vi "GDSString_ParseTextBasedCode.vi"(8 "error in (no error)":errorcluster, 11 "TextIn":string="public interface IGoldMembership\n    {\n        decimal GetDiscount(decimal amount);\n        bool IsShippingFree { get; set; }\n    }\n \npublic class GoldMembership : IGoldMembership\n    {\n        public GoldMembership(string userName)\n        {\n            // get gold member profile of this user\n \n            IsShippingFree = true;\n        }\n \n        public bool IsShippingFree { get; set; }\n \n        public decimal GetDiscount(decimal amount)\n        {\n            decimal discount = 100;\n \n            //calculate discount\n \n            return discount;\n        }\n    }\n \npublic class NullGoldMembership : IGoldMembership\n    {\n        public NullGoldMembership()\n        {\n            IsShippingFree = false;\n        }\n \n        public decimal GetDiscount(decimal amount)\n        {\n            return 0;\n        }\n \n        public bool IsShippingFree { get; set; }\n    }\n \npublic class GoldMembershipController\n    {\n        public static IGoldMembership GetProfile(Account account)\n        {\n            // if this account has gold membership \n            // return profile else return null\n \n            if (account.Type == \"GoldMember\")\n            {\n                return new GoldMembership(account.UserName);\n            }\n            else\n            {\n                return new NullGoldMembership();\n            }\n        }\n    }\n") -> (0 "error out":errorcluster, 1 "EnumsOusideClass":T1[](array[typedef])=[{"Name"="Orientation", "AccessScope"=enum."public", "Modifiers"=[], "Items"=["TOP", "LEFT"], "Documentation"=""}, {"Name"="Range", "AccessScope"=enum."public", "Modifiers"=[], "Items"=["Max", "Min"], "Documentation"=""}, {"Name"="CarOptions", "AccessScope"=enum."public", "Modifiers"=[], "Items"=["SunRoof", "Spoiler", "FogLights", "TintedWindows"], "Documentation"=""}], 2 "StructsOusideClass":T4[](array[typedef])=[{"Name"="", "AccessScope"=enum."public", "Modifiers"=[], "Items"=[], "Documentation"=""}], 3 "Classes":T7[](array[typedef])=[{"ClassName"="EmailErrorHandler", "AccessScope"=enum."public", "Modifiers"=[], "ClassDocumentation"="public", "Methods"=[{"ReturnType"={"Name"="", "DataType"=enum."UINT8", "ArrayDim"=0, "CtrlPath"=path "", "DataTypeString"="", "AccessScope"=enum."public", "InitialData"=variant}, "MethodName"="", "AccessScope"=enum."public", "Modifiers"=[], "MethodDocumentation"="", "MethodContent"="", "MethodArguments"=[], "GetProperty"={"Active"=FALSE, "AccessScope"=enum."public", "Code"=""}, "SetProperty"={"Active"=FALSE, "AccessScope"=enum."public", "Code"=""}}, {"ReturnType"={"Name"="", "DataType"=enum."UINT8", "ArrayDim"=0, "CtrlPath"=path "", "DataTypeString"="", "AccessScope"=enum."public", "InitialData"=variant}, "MethodName"="", "AccessScope"=enum."public", "Modifiers"=[], "MethodDocumentation"="", "MethodContent"="", "MethodArguments"=[], "GetProperty"={"Active"=FALSE, "AccessScope"=enum."public", "Code"=""}, "SetProperty"={"Active"=FALSE, "AccessScope"=enum."public", "Code"=""}}, {"ReturnType"={"Name"="", "DataType"=enum."UINT8", "ArrayDim"=0, "CtrlPath"=path "", "DataTypeString"="", "AccessScope"=enum."public", "InitialData"=variant}, "MethodName"="", "AccessScope"=enum."public", "Modifiers"=[], "MethodDocumentation"="", "MethodContent"="", "MethodArguments"=[], "GetProperty"={"Active"=FALSE, "AccessScope"=enum."public", "Code"=""}, "SetProperty"={"Active"=FALSE, "AccessScope"=enum."public", "Code"=""}}, {"ReturnType"={"Name"="", "DataType"=enum."UINT8", "ArrayDim"=0, "CtrlPath"=path "", "DataTypeString"="", "AccessScope"=enum."public", "InitialData"=variant}, "MethodName"="", "AccessScope"=enum."public", "Modifiers"=[], "MethodDocumentation"="", "MethodContent"="", "MethodArguments"=[], "GetProperty"={"Active"=FALSE, "AccessScope"=enum."public", "Code"=""}, "SetProperty"={"Active"=FALSE, "AccessScope"=enum."public", "Code"=""}}], "ParentClasses"=[{"ClassName"="IErrorHandler", "ClassType"=enum."Undefined"}], "ClassType"=enum."Class", "Owner"="", "OwnerType"=enum."NoOwner", "Generics"=[], "Attributes"=[{"Name"="settings", "DataType"=enum."Other", "ArrayDim"=0, "CtrlPath"=path "", "DataTypeString"="EmailErrorHandlerParms", "AccessScope"=enum."private", "InitialData"=variant(string "")}], "Enums"=[], "Structs"=[]}, {"ClassName"="EmailErrorHandlerParms", "AccessScope"=enum."public", "Modifiers"=[], "ClassDocumentation"="", "Methods"=[{"ReturnType"={"Name"="", "DataType"=enum."UINT8", "ArrayDim"=0, "CtrlPath"=path "", "DataTypeString"="", "AccessScope"=enum."public", "InitialData"=variant}, "MethodName"="", "AccessScope"=enum."public", "Modifiers"=[], "MethodDocumentation"="", "MethodContent"="", "MethodArguments"=[], "GetProperty"={"Active"=FALSE, "AccessScope"=enum."public", "Code"=""}, "SetProperty"={"Active"=FALSE, "AccessScope"=enum."public", "Code"=""}}, {"ReturnType"={"Name"="", "DataType"=enum."UINT8", "ArrayDim"=0, "CtrlPath"=path "", "DataTypeString"="", "AccessScope"=enum."public", "InitialData"=variant}, "MethodName"="", "AccessScope"=enum."public", "Modifiers"=[], "MethodDocumentation"="", "MethodContent"="", "MethodArguments"=[], "GetProperty"={"Active"=FALSE, "AccessScope"=enum."public", "Code"=""}, "SetProperty"={"Active"=FALSE, "AccessScope"=enum."public", "Code"=""}}, {"ReturnType"={"Name"="", "DataType"=enum."UINT8", "ArrayDim"=0, "CtrlPath"=path "", "DataTypeString"="", "AccessScope"=enum."public", "InitialData"=variant}, "MethodName"="", "AccessScope"=enum."public", "Modifiers"=[], "MethodDocumentation"="", "MethodContent"="", "MethodArguments"=[], "GetProperty"={"Active"=FALSE, "AccessScope"=enum."public", "Code"=""}, "SetProperty"={"Active"=FALSE, "AccessScope"=enum."public", "Code"=""}}, {"ReturnType"={"Name"="", "DataType"=enum."UINT8", "ArrayDim"=0, "CtrlPath"=path "", "DataTypeString"="", "AccessScope"=enum."public", "InitialData"=variant}, "MethodName"="", "AccessScope"=enum."public", "Modifiers"=[], "MethodDocumentation"="", "MethodContent"="", "MethodArguments"=[], "GetProperty"={"Active"=FALSE, "AccessScope"=enum."public", "Code"=""}, "SetProperty"={"Active"=FALSE, "AccessScope"=enum."public", "Code"=""}}, {"ReturnType"={"Name"="", "DataType"=enum."UINT8", "ArrayDim"=0, "CtrlPath"=path "", "DataTypeString"="", "AccessScope"=enum."public", "InitialData"=variant}, "MethodName"="", "AccessScope"=enum."public", "Modifiers"=[], "MethodDocumentation"="", "MethodContent"="", "MethodArguments"=[], "GetProperty"={"Active"=FALSE, "AccessScope"=enum."public", "Code"=""}, "SetProperty"={"Active"=FALSE, "AccessScope"=enum."public", "Code"=""}}], "ParentClasses"=[], "ClassType"=enum."Class", "Owner"="EmailErrorHandler", "OwnerType"=enum."Class", "Generics"=[], "Attributes"=[], "Enums"=[], "Structs"=[]}])   [LabVIEW 2020]
uses:
  GDSString_ClassDescriptionType.ctl
  GDSString_AccessScopeModifierType.ctl
  GDSString_ModifierType.ctl
  GDSString_MethodDescriptionType.ctl
  CommonVIs/CommonVIs_AttributeType.ctl
  CommonVIs/CommonVIs_AttributeDataType.ctl
  CommonVIs/CommonVIs_PropertyType.ctl
  GDSString_ClassParentType.ctl
  GDSString_ClassType.ctl
  GDSString_ClassOwnerType.ctl
  CommonVIs/CommonVIs_EnumType.ctl
  CommonVIs/CommonVIs_StructType.ctl
panel:
  # "using System;\n\nnamespace TutlaneExamples\n{\n    class Users\n    {\n       // Declare an array\n       private string[] arr = new string[3];\n       // Define the indexer\n       public string this[int i]\n       {\n          get { return arr[i]; }\n          set { arr[i] = value; }\n       }\n    }\n    class Program\n    {\n       static void Main(string[] args)\n       {\n          Users ulist = new Users();\n          ulist[0] = \"Suresh Dasari\";\n          ulist[1] = \"Rohini Alavala\";\n          ulist[2] = \"Trishika Dasari\";\n          for (int i = 0; i < 3; i++)\n          {\n             Console.WriteLine(ulist[i]);\n          }\n          Console.ReadLine();\n       }\n    }\n}"
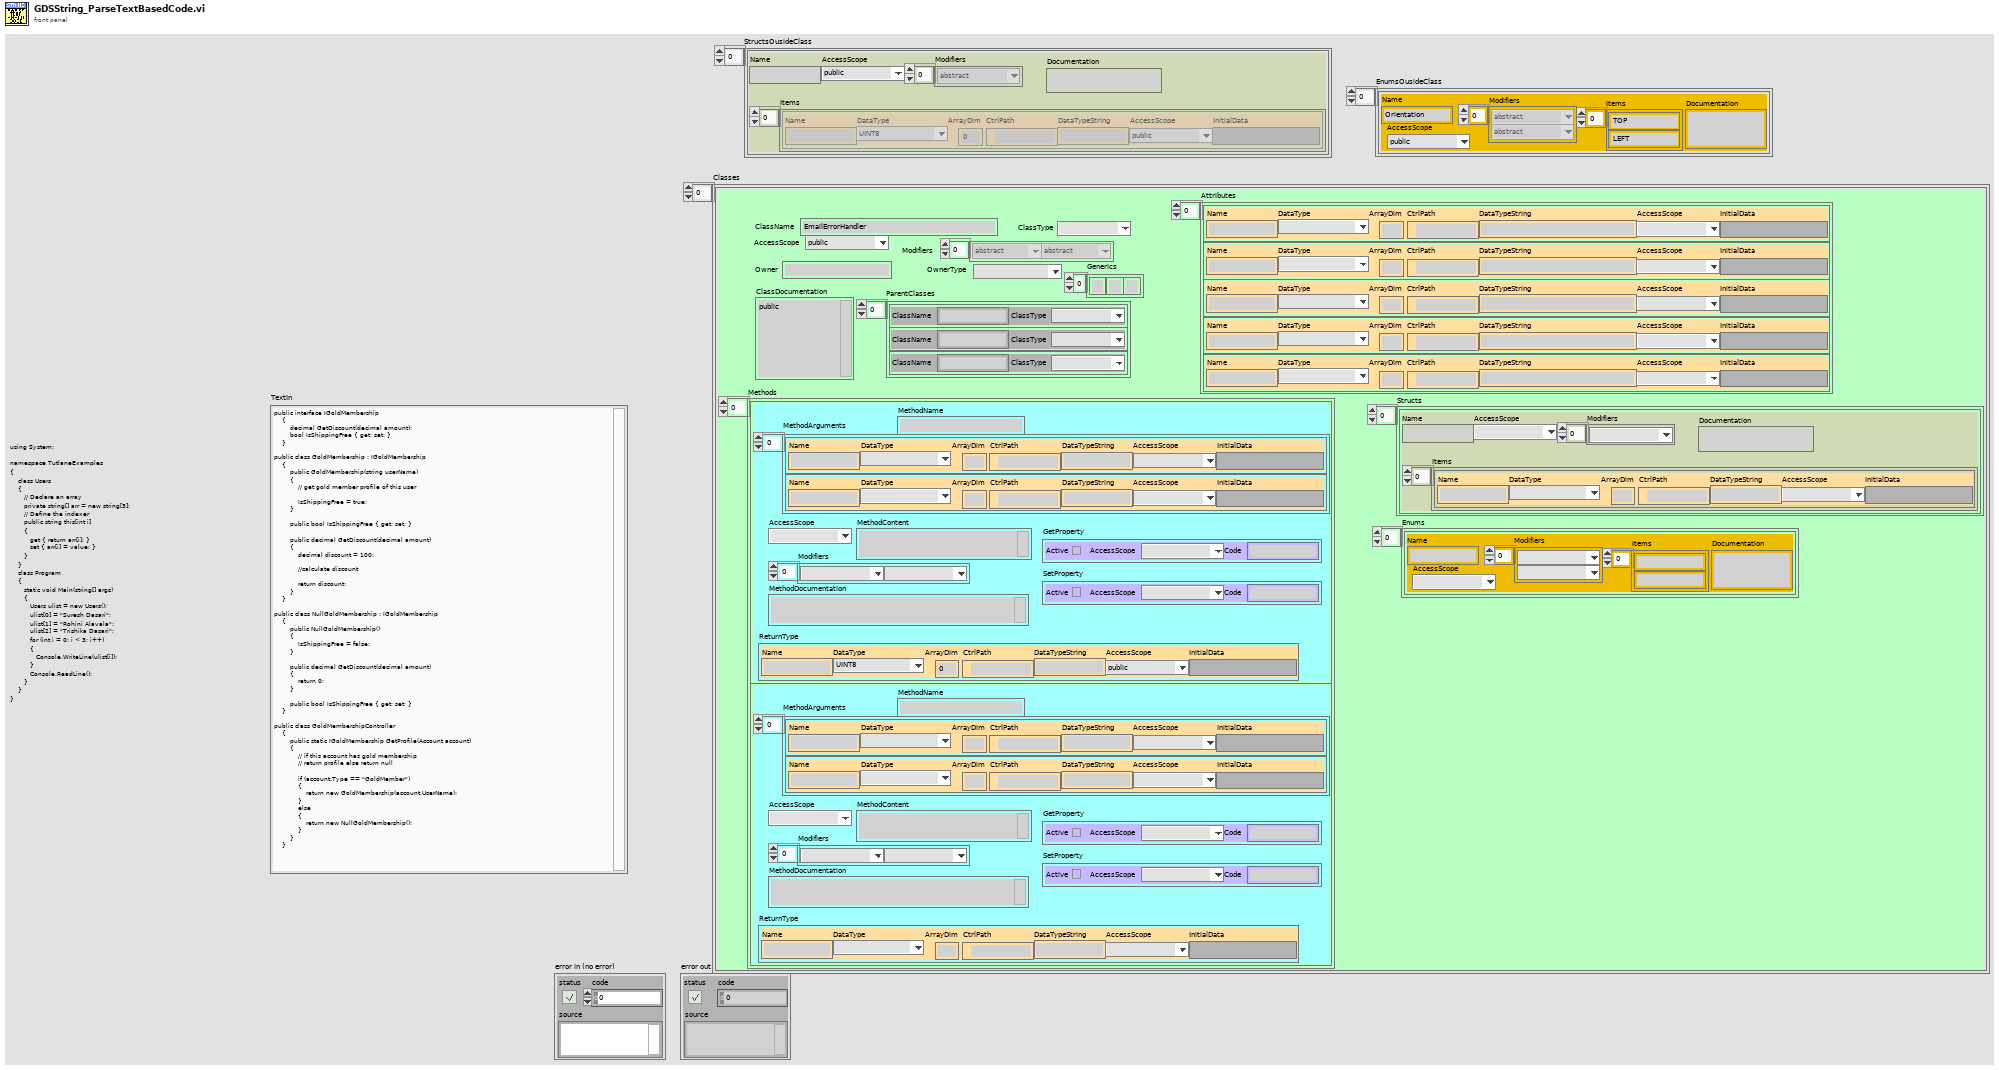
[diagram p1: front panel]
types:
  T1 = typedef "CommonVIs_EnumType.ctl" = cluster{"Name":string, "AccessScope":T2, "Modifiers":T3[], "Items":string[], "Documentation":string}
  T2 = typedef "GDSString_AccessScopeModifierType.ctl" = enum16{"public", "private", "protected", "internal"}
  T3 = typedef "GDSString_ModifierType.ctl" = enum16{"abstract", "static", "final", "synchronized", "strictfp", "async", "const", "event", "extern", "new", "native ", "override", "partial", "readonly", "sealed", "unsafe", "virtual", "volatile"}
  T4 = typedef "CommonVIs_StructType.ctl" = cluster{"Name":string, "AccessScope":T2, "Modifiers":T3[], "Items":T5[], "Documentation":string}
  T5 = typedef "CommonVIs_AttributeType.ctl" = cluster{"Name":string, "DataType":T6, "ArrayDim":i32, "CtrlPath":path, "DataTypeString":string, "AccessScope":T2, "InitialData":variant}
  T6 = typedef "CommonVIs_AttributeDataType.ctl" = enum16{"UINT8", "INT8", "UINT16", "INT16", "UINT32", "INT32", "UINT64", "INT64", "SGL", "DBL", "EXT", "CSG", "CDB", "CXT", "TimeStamp", "STRING", "PATH", "BOOL", "ENUM", "RefNum", "VIRefNum", "LabVIEW Class", "Cluster", "Variant", "TypeDef", "Waveform", "LabVIEW Object", "Other", "void", "Set", "Map"}
  T7 = typedef "GDSString_ClassDescriptionType.ctl" = cluster{"ClassName":string, "AccessScope":T2, "Modifiers":T3[], "ClassDocumentation":string, "Methods":T8[], "ParentClasses":T10[], "ClassType":T11, "Owner":string, "OwnerType":T12, "Generics":string[], "Attributes":T5[], "Enums":T1[], "Structs":T4[]}
  T8 = typedef "GDSString_MethodDescriptionType.ctl" = cluster{"ReturnType":T5, "MethodName":string, "AccessScope":T2, "Modifiers":T3[], "MethodDocumentation":string, "MethodContent":string, "MethodArguments":T5[], "GetProperty":T9, "SetProperty":T9}
  T9 = typedef "CommonVIs_PropertyType.ctl" = cluster{"Active":bool, "AccessScope":T2, "Code":string}
  T10 = typedef "GDSString_ClassParentType.ctl" = cluster{"ClassName":string, "ClassType":T11}
  T11 = typedef "GDSString_ClassType.ctl" = enum16{"Undefined", "Class", "Interface"}
  T12 = typedef "GDSString_ClassOwnerType.ctl" = enum16{"NoOwner", "Class", "Package/NameSpace"}
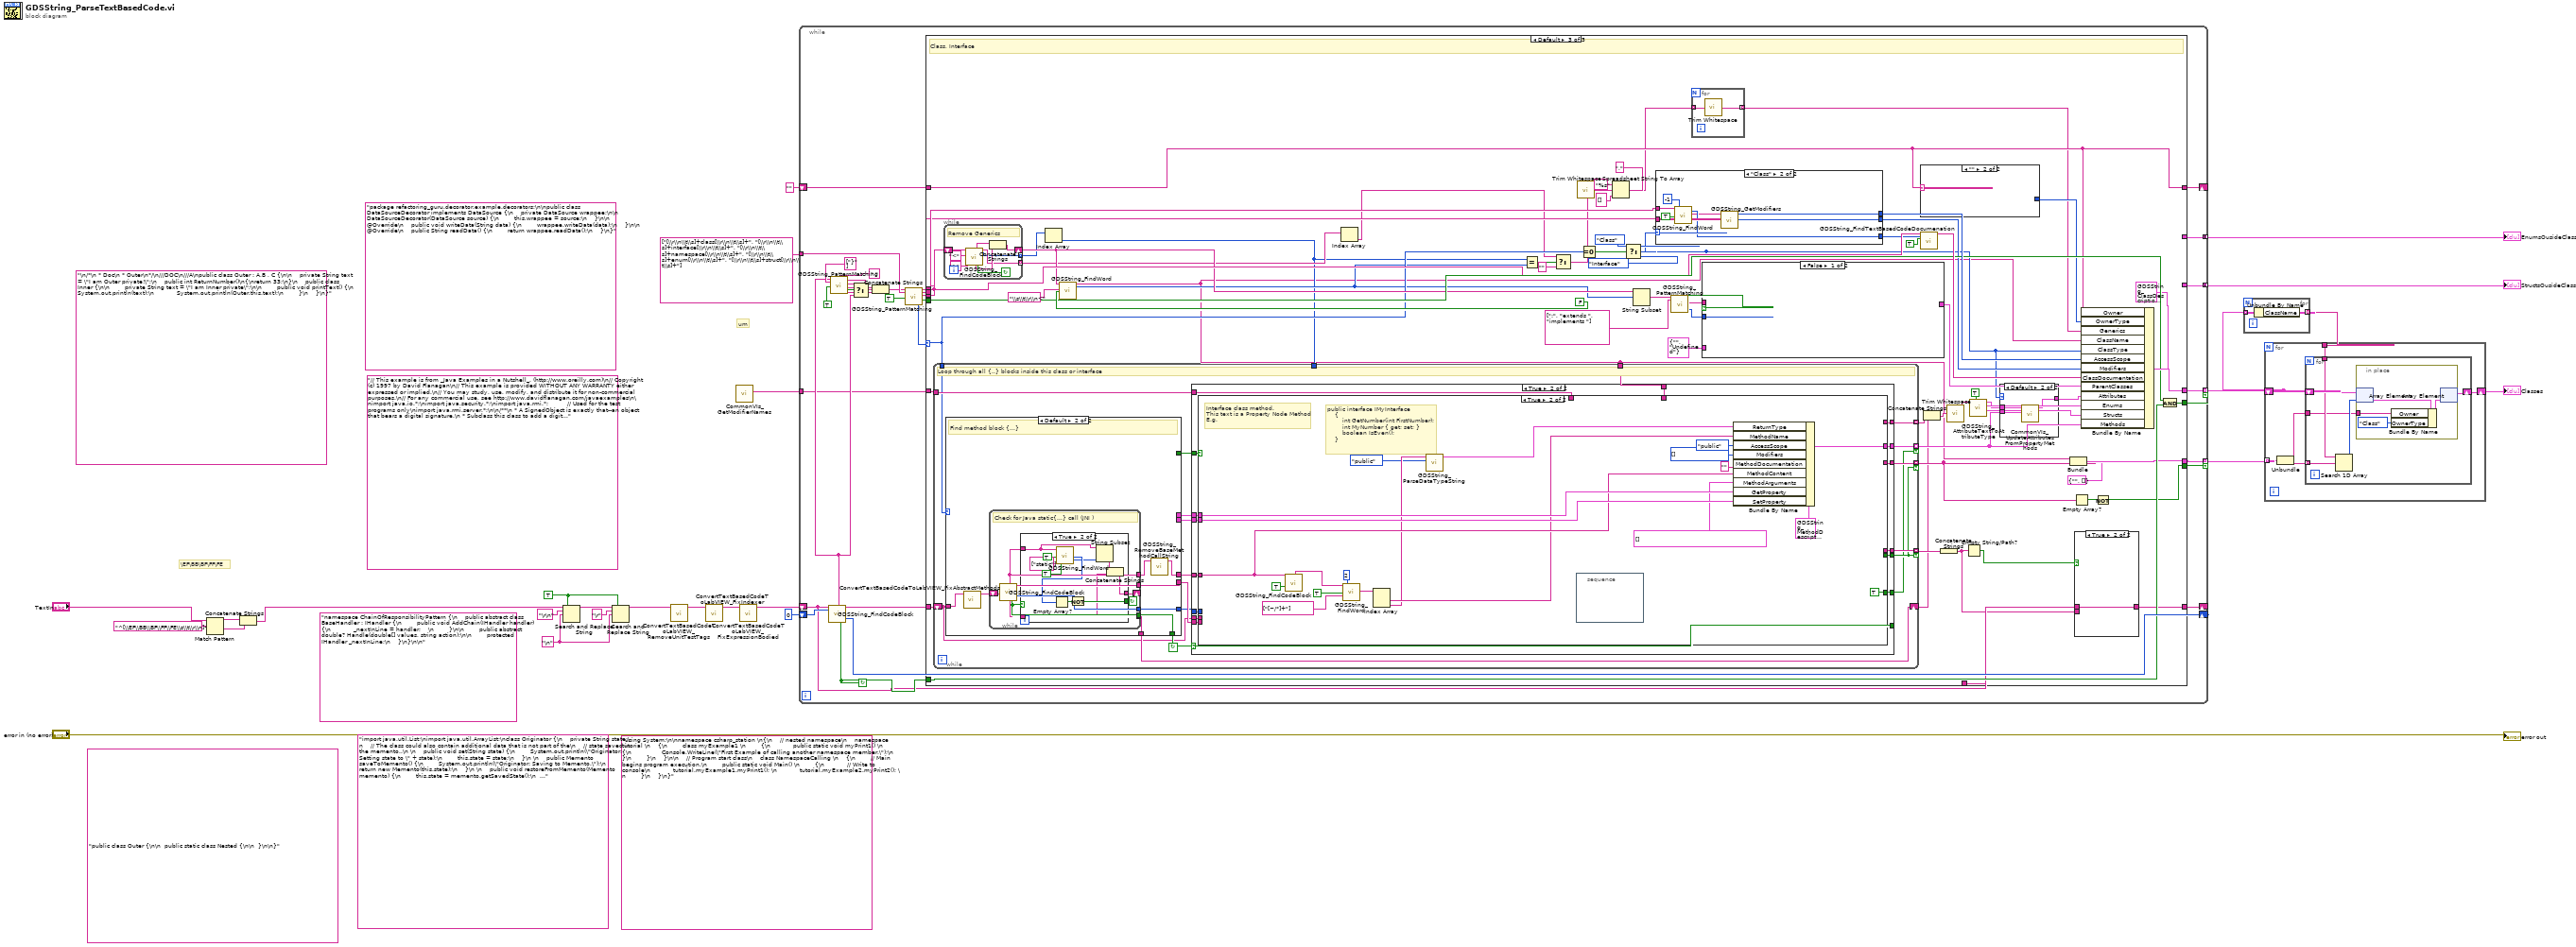
[diagram p0: block diagram]
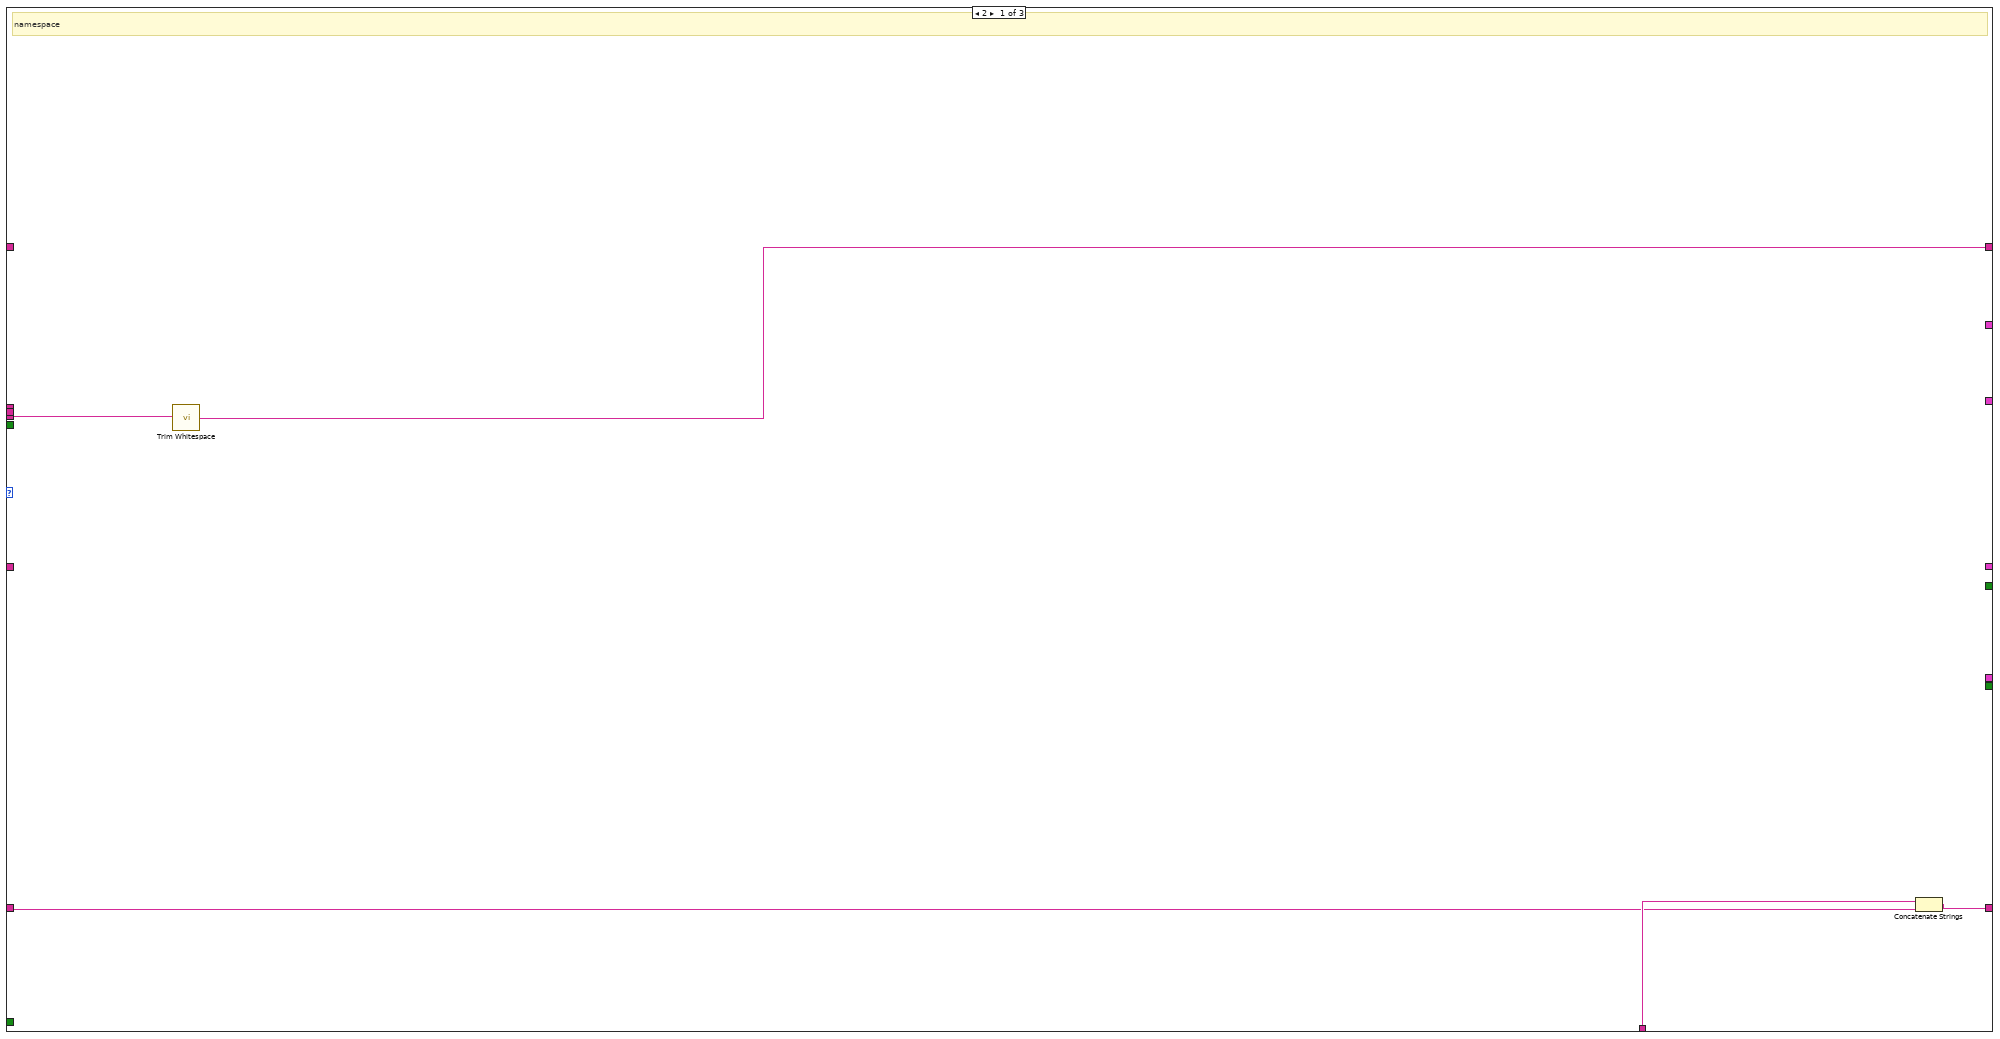
[diagram p2: hidden frame]
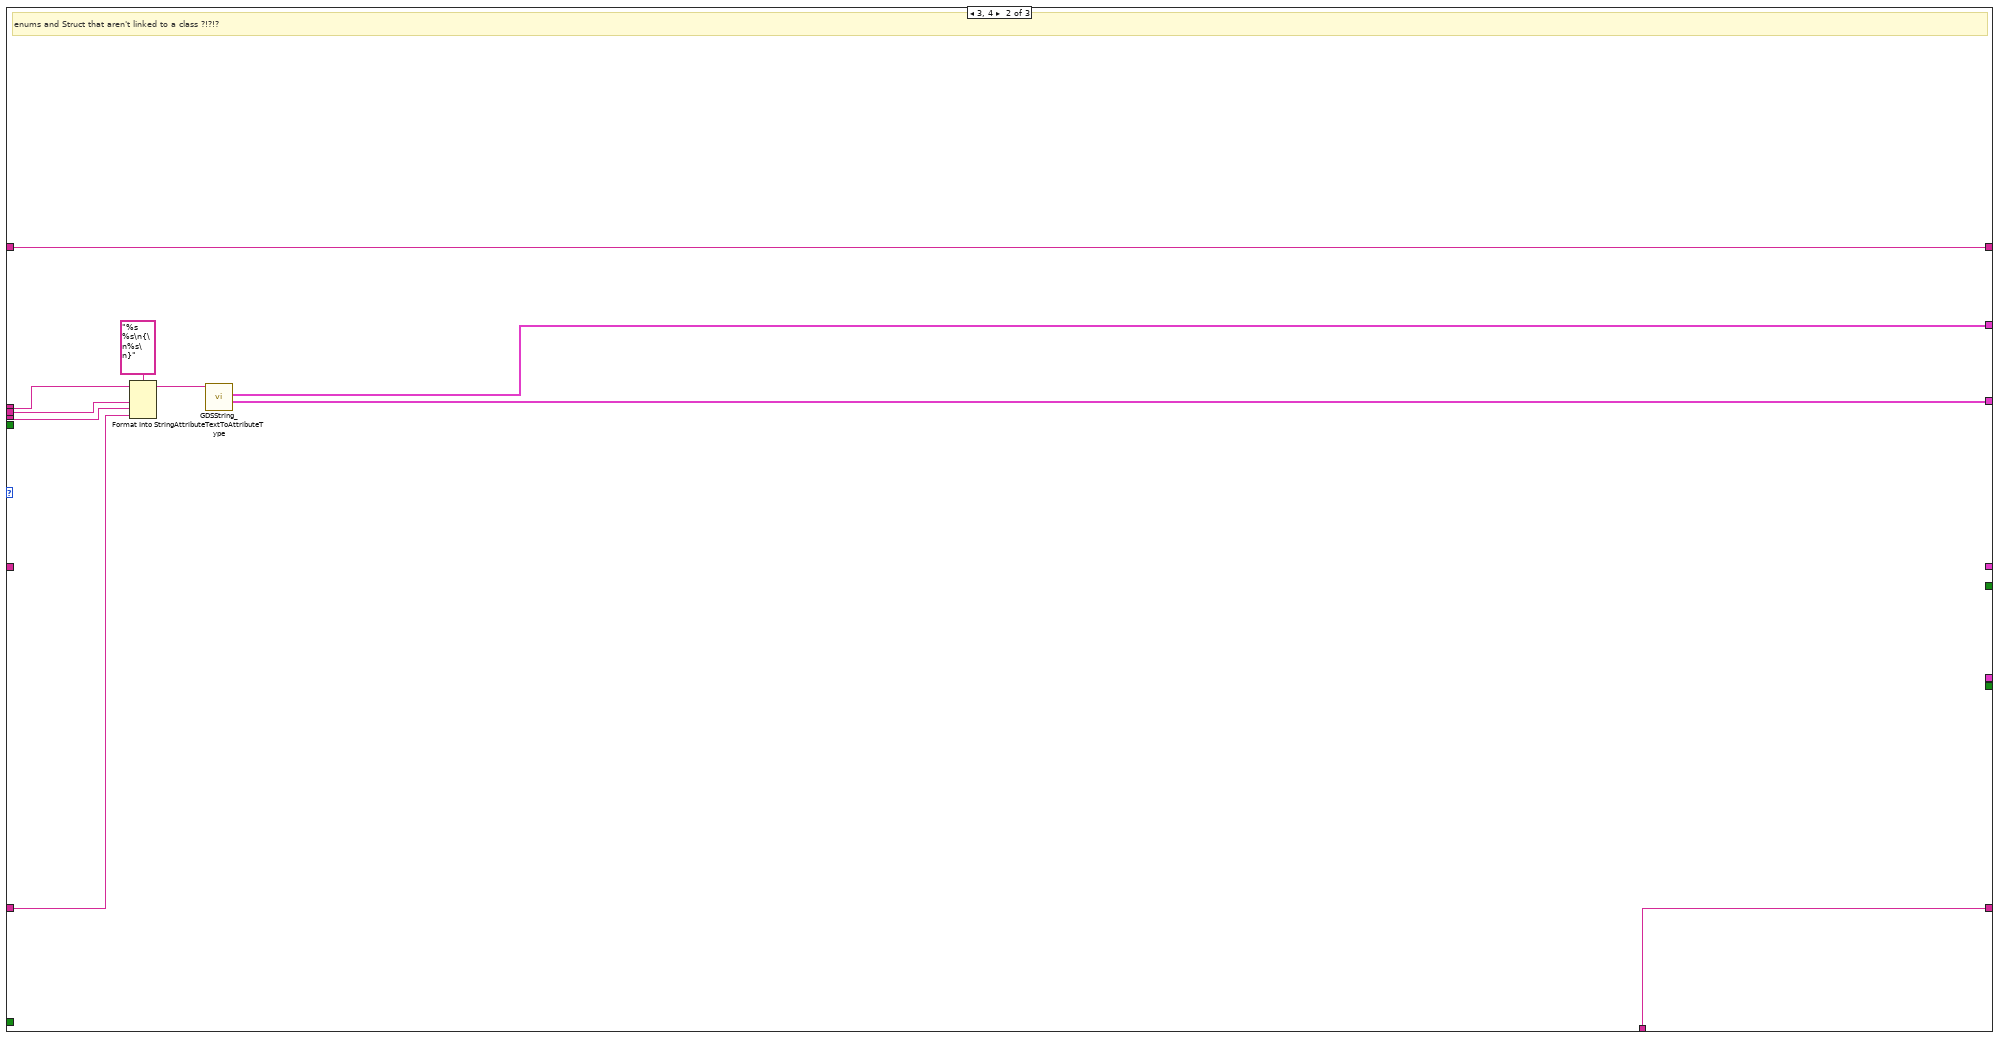
[diagram p3: hidden frame]
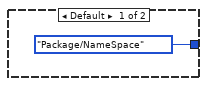
[diagram p5: hidden frame]
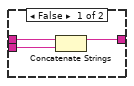
[diagram p6: hidden frame]
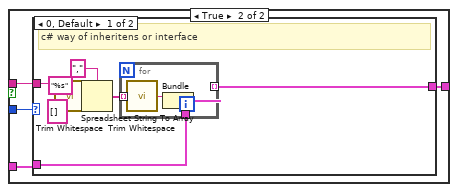
[diagram p7: hidden frame]
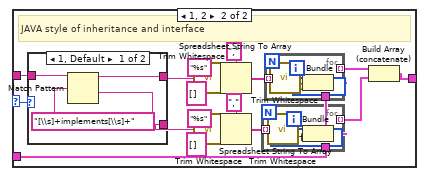
[diagram p8: hidden frame]
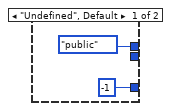
[diagram p10: hidden frame]
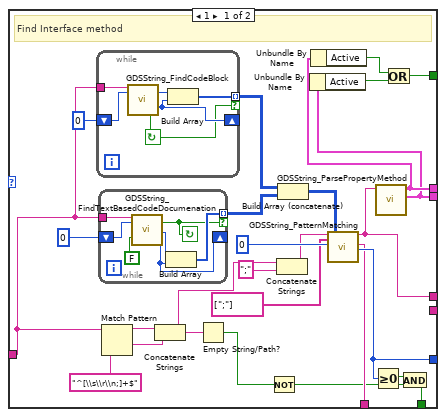
[diagram p11: hidden frame]
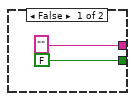
[diagram p12: hidden frame]
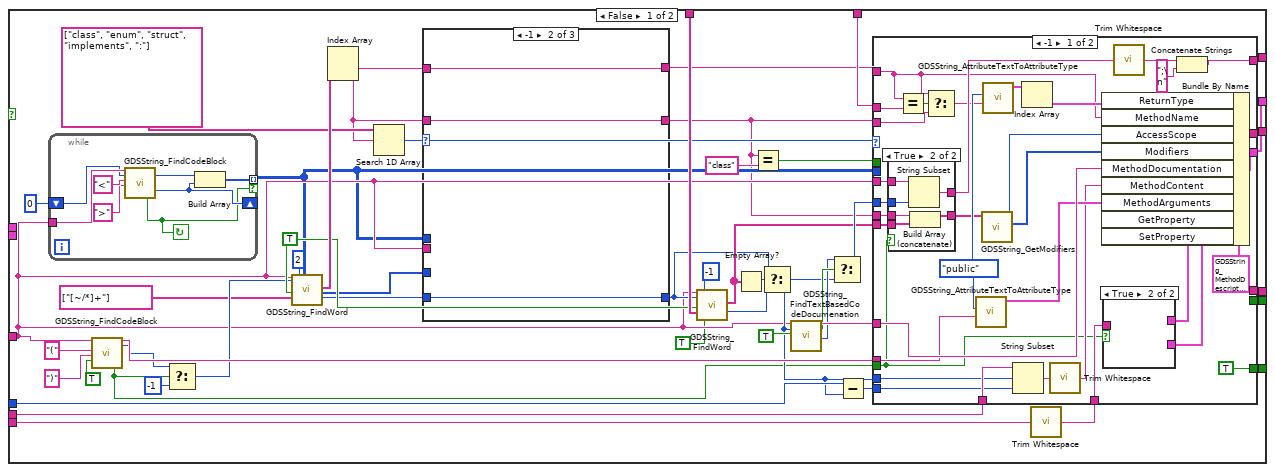
[diagram p14: hidden frame]
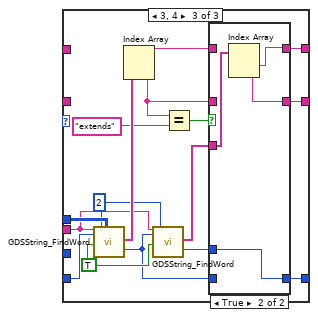
[diagram p16: hidden frame]
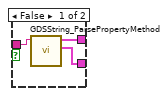
[diagram p19: hidden frame]
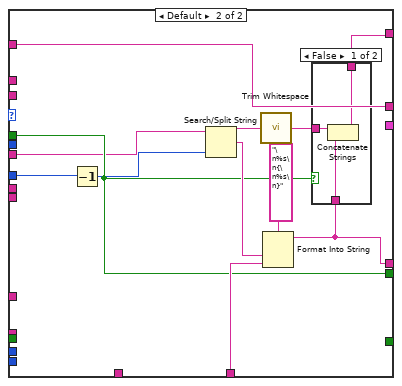
[diagram p20: hidden frame]
diagram:
  (unwired) "namespace ChainOfResponsibilityPattern {\n    public abstract class BaseHandler : IHandler {\n        public void AddChain(IHandler handler) {\n            _nextInLine = handler;    \n        }\n\n        public abstract double? Handle(double[] values, string action);\n\n        protected IHandler _nextInLine;\n    }\n}\n\n" ("search string")
  (unwired) "package refactoring_guru.decorator.example.decorators;\n\npublic class DataSourceDecorator implements DataSource {\n    private DataSource wrappee;\n\n    DataSourceDecorator(DataSource source) {\n        this.wrappee = source;\n    }\n\n    @Override\n    public void writeData(String data) {\n        wrappee.writeData(data);\n    }\n\n    @Override\n    public String readData() {\n        return wrappee.readData();\n    }\n}" ("text")
  (unwired) "using System;\n\nnamespace csharp_station \n{\n    // nested namespace\n    namespace tutorial \n    {\n        class myExample1 \n        {\n            public static void myPrint1() \n            {\n                Console.WriteLine(\"First Example of calling another namespace member.\");\n            }\n        }\n    }\n\n    // Program start class\n    class NamespaceCalling \n    {\n        // Main begins program execution.\n        public static void Main() \n        {\n            // Write to console\n            tutorial.myExample1.myPrint1(); \n            tutorial.myExample2.myPrint2(); \n        }\n    }\n}" ("text")
  (unwired) "public class Outer {\n\n  public static class Nested {\n\n  }\n\n}" ("text")
  (unwired) "import java.util.List;\nimport java.util.ArrayList;\nclass Originator {\n    private String state;\n    // The class could also contain additional data that is not part of the\n    // state saved in the memento..\n \n    public void set(String state) {\n        System.out.println(\"Originator: Setting state to \" + state);\n        this.state = state;\n    }\n \n    public Memento saveToMemento() {\n        System.out.println(\"Originator: Saving to Memento.\");\n        return new Memento(this.state);\n    }\n \n    public void restoreFromMemento(Memento memento) {\n        this.state = memento.getSavedState();\n        System.out.println(\"Originator: State after restoring from Memento: \" + state);\n    }\n \n    public static class Memento {\n        private final String state;\n \n        public Memento(String stateToSave) {\n            state = stateToSave;\n        }\n \n        public String getSavedState() {\n            return state;\n        }\n    }\n}\n \nclass Caretaker {\n    public static void main(String[] args) {\n        List<Originator.Memento> savedStates = new ArrayList<Originator.Memento>();\n \n        Originator originator = new Originator();\n        originator.set(\"State1\");\n        originator.set(\"State2\");\n        savedStates.add(originator.saveToMemento());\n        originator.set(\"State3\");\n        // We can request multiple mementos, and choose which one to roll back to.\n        savedStates.add(originator.saveToMemento());\n        originator.set(\"State4\");\n \n        originator.restoreFromMemento(savedStates.get(1));   \n    }\n}" ("text")
  (unwired) "// This example is from _Java Examples in a Nutshell_. (http://www.oreilly.com)\n// Copyright (c) 1997 by David Flanagan\n// This example is provided WITHOUT ANY WARRANTY either expressed or implied.\n// You may study, use, modify, and distribute it for non-commercial purposes.\n// For any commercial use, see http://www.davidflanagan.com/javaexamples\n\nimport java.io.*;\nimport java.security.*;\nimport java.rmi.*;          // Used for the test programs only\nimport java.rmi.server.*;\n\n/**\n * A SignedObject is exactly that--an object that bears a digital signature.\n * Subclass this class to add a digital signature to any class you want.\n * Note, however, that the signature is computed using serialization, so only\n * the serializable, non-transient fields of a subclass are included in\n * the signature computation.\n **/\npublic class SignedObject implements Serializable {\n  protected String signername;               // Who is doing the signing\n  protected String algorithm;                // What algorithm to use.\n  private byte[] signature;                  // The bytes of the signature\n  transient private boolean signing = false; // A flag used below.\n\n  /**\n   * This method computes a digital signature for the current state of the\n   * object, excluding the signature-related state of this class.\n   * That is, the signature is based only on the state of the subclasses.\n   * The arguments specify who is signing the object, and what digital \n   * signature algorithm to use.\n   * \n   * Note that no other threads should be modifying the object while\n   * this computation is being performed.  If a subclass will be used in a \n   * multi-threaded environment, this means that methods of the subclass\n   * that modify its state should be synchronized like this one is.\n   **/\n  public synchronized void sign(String signername, String algorithm) \n       throws IOException, InvalidKeyException, \n         SignatureException, NoSuchAlgorithmException \n  {\n    // Save the arguments for use by verify()\n    this.signername = signername;\n    this.algorithm = algorithm;\n\n    // Get a Signature object to compute the signature with\n    Signature s = Signature.getInstance(algorithm);\n\n    // Get a Signer object representing the signer\n    Signer signer = \n      (Signer)IdentityScope.getSystemScope().getIdentity(signername);\n\n    // Initialize the Signature object using the PrivateKey of the Signer\n    s.initSign(signer.getPrivateKey());\n\n    // Create an ObjectOutputStream that writes its output to a \n    // ByteArrayStream.  This is how we capture the state of the object\n    // so that it can be signed.\n    ByteArrayOutputStream bout = new ByteArrayOutputStream();\n    ObjectOutputStream out = new ObjectOutputStream(bout);\n\n    // Now serialize the object, capturing its state.  We have to set a flag\n    // before we do this, so that the signer name, algorithm, and signature\n    // itself are not included in this serialized state.  See writeObject()\n    // below to see how this works.\n    signing = true;\n    out.writeObject(this);\n    signing = false;\n\n    // Now tell the Signature object about the bytes of serialized state\n    // that were stored by the ByteArrayOutputStream\n    s.update(bout.toByteArray());\n\n    // And finally, compute the signature\n    this.signature = s.sign();\n  }\n\n  /** A simpler version of sign(), that defaults to using the DSA algorithm */\n  public synchronized void sign(String signername) \n       throws IOException, InvalidKeyException, \n         SignatureException, NoSuchAlgorithmException {\n    sign(signername, \"DSA\");\n  }\n\n  /**\n   * This method verifies the signature of any SignedObject subclass.\n   * It works much like the sign() method, and is also synchronized.\n   **/\n  public synchronized boolean verify() \n       throws IOException, InvalidKeyException,\n         SignatureException, NoSuchAlgorithmException\n  {\n    // Make sure the object is actually signed.\n    if (signature == null) \n      throw new SignatureException(\"Object is not signed\");\n\n    // Get the signature, signer and public key, and initialize, like above,\n    // except that this time use a PublicKey instead of a PrivateKey\n    Signature s = Signature.getInstance(algorithm);\n    Identity signer = \n      (Identity)IdentityScope.getSystemScope().getIdentity(signername);\n    s.initVerify(signer.getPublicKey());\n\n    // Create streams and capture the current state of the object \n    // (excluding the signature bytes themselves) in a byte array\n    ByteArrayOutputStream bout = new ByteArrayOutputStream();\n    ObjectOutputStream out = new ObjectOutputStream(bout);\n    signing = true;\n    out.writeObject(this);\n    signing = false;\n\n    // Pass state of the object to the Signature, and verify the stored\n    // signature bytes against that state.  Return the result of verification.\n    s.update(bout.toByteArray());\n    return s.verify(this.signature);\n  }\n\n  /**\n   * When the contents of the object change, the signature becomes invalid.\n   * When this happens, the signature should be erased, because validation\n   * is guaranteed to fail.\n   **/\n  public void removeSignature() { \n    signature = null; signername = null; algorithm = null; \n  }\n\n  /**\n   * This method is invoked to allow custom serialization.\n   * We only write out our signature-related state when we are not computing\n   * or verifying a signature.  When we are computing or verifying, only our\n   * subclass state gets written out.  If we don't do this, verification will\n   * fail because the signature[] array will obviously be different on\n   * verification than it is when the signature is generated.\n   **/\n  private void writeObject(ObjectOutputStream out) throws IOException {\n    if (!signing) out.defaultWriteObject();\n  }\n}\n\n/**\n * This class is a simple SignedObject subclass.\n * This and the following interface and classes are used to test SignedObject.\n **/\nclass SignedString extends SignedObject {\n  public String s;\n  public SignedString(String s) { this.s = s; }\n}\n\n/**\n * This interface extends Remote.  It is part of an RMI example using our\n * SignedString class above.\n **/\ninterface RemoteSignedString extends Remote {\n  public SignedString getString() throws RemoteException;\n}\n\n/**\n * This is a simple RMI server class and a program to start and register the\n * server.  The server creates a SignedString object, signs it, and then \n * exports it to clients through the RemoteSignedString getString() method.\n **/\nclass SignedStringServer extends UnicastRemoteObject \n                         implements RemoteSignedString \n{\n  SignedString s;  // The state of the server object\n\n  /** The constructor.  Initialize the SignedString */\n  public SignedStringServer(SignedString s) throws RemoteException {this.s=s;}\n\n  /** This is the remote method exported by the server */\n  public SignedString getString() throws RemoteException { return s; }\n  \n  /** The main program that creates and registers the server object */\n  public static void main(String[] args) \n       throws NoSuchAlgorithmException, InvalidKeyException, \n         IOException, SignatureException\n  {\n    SignedString ss = new SignedString(args[0]);         // create object\n    ss.sign(args[1]);                                    // sign it\n    SignedStringServer sss = new SignedStringServer(ss); // start server\n    Naming.rebind(\"SignedStringServer\", sss);            // register server\n    System.out.println(\"Ready for clients\");             // up and running!\n  }\n}\n\n/**\n * This class is a client that connects to a RemoteSignedString server and\n * calls the getString() method to obtain a SignedString.  It then verifies\n * the signature of the object that it has just downloaded over a network\n * from an entirely different Java VM.  The client takes an optional hostname\n * argument on the command line.\n **/\nclass SignedStringClient {\n  public static void main(String[] args)\n       throws NoSuchAlgorithmException, InvalidKeyException, \n         IOException, SignatureException, NotBoundException\n  {\n    // Look up the server\n    RemoteSignedString rss = \n      (RemoteSignedString) Naming.lookup(\"rmi://\" + \n                                         ((args.length>0)?args[0]:\"\") +\n                                         \"/SignedStringServer\"); \n\n    // Invoke a remote method of the server to get a SignedString\n    SignedString ss = rss.getString();\n\n    // Now verify the signature on that SignedString.\n    if (ss.verify()) System.out.println(\"Verified SignedString: \" + ss.s);\n    else System.out.println(\"SignedString failed verification\");\n  }\n}\n" ("text")
  w10 = TRUE ("replace all? (F)")
  w22 = "\n" ("search string")
  (unwired) "\n/*\n * Doc\n * Outer\n*/\n///DOC\n///A\npublic class Outer : A,B , C {\n\n    private String text = \"I am Outer private!\";\n    public int ReturnNumber()\n{\nreturn 33;\n}\n    public class Inner {\n\n        private String text = \"I am Inner private\";\n\n        public void printText() {\n            System.out.println(text);\n            System.out.println(Outer.this.text);\n        }\n    }\n}" ("text")
  # "\\EF\\BB\\BF\\FF\\FE"
  # "um"
  n1 = Match Pattern(string="TextIn", regular expression="^[\\EF\\BB\\BF\\FF\\FE\\s\\t\\r\\n]+") -> (before substring=w8:string, after substring=w7:string)  [unwired: 1 in, 2 out]
  n2 = Concatenate Strings(w8, w7) -> (w5:string)
  n3 = Search and Replace String(replace all?=w10, input string=w5, search string="\r\n", replace string=w22) -> (result string=w25:string)  [unwired: 4 in, 3 out]
  n4 = Search and Replace String(replace all?=w10, input string=w25, search string="\r", replace string=w22) -> (result string=w2:string)  [unwired: 4 in, 3 out]
  n5 = call "ConvertTextBasedCodeToLabVIEW_RemoveUnitTestTags.vi"("TextIn"=w2) -> ("TextOut"=w1:string)  [unwired: 10 in]
  n6 = call "ConvertTextBasedCodeToLabVIEW_FixIndexer.vi"("IndexerTextIn"=w1) -> ("MofifiedIndexerTextOut"=w4:string)  [unwired: 10 in]
  n7 = call "CommonVIs_GetModifierNames.vi"() -> ("AllModifiers"=w13:string[])  [unwired: 9 in, 2 out]
  n8 = call "ConvertTextBasedCodeToLabVIEW_FixExpressionBodied.vi"("Expression-bodiedTextIn"=w4) -> ("ModifiedExpression-bodiedTextOut"=w3:string)  [unwired: 10 in]
  n9 = while {
    tunnel: w13 -> [w39]
    shift-right: [w53] -> _
    shift-left: 0 ("GetNext-X_Words(1,-1=All)") -> [w54]
    tunnel: [w52] -> w19 mode=indexing if=w43
    shift-right: [w37] -> _
    shift-left: w3 -> [w38]
    tunnel: [w36] -> w20 mode=indexing if=w35
    tunnel: string[] ["[\\r\\n\\t\\s]+class[\\r\\n\\t\\s]+", "[\\r\\n\\t\\s]+interface[\\r\\n\\t\\s]+", "[\\r\\n\\t\\s]+namespace[\\r\\n\\t\\s]+", "[\\r\\n\\t\\s]+enum[\\r\\n\\t\\s]+", "[\\r\\n\\t\\s]+struct[\\r\\n\\t\\s]+"] -> [w34]
    shift-right: [w31] -> _
    shift-left: "" ("trimmed string") -> [w30]
    tunnel: [w27] -> w11 mode=concatenating
    tunnel: [w26] -> w12 mode=concatenating
    stop <- w44 continue-if-true
    n10 = call "GDSString_FindCodeBlock.vi"("Text"=w38, "StringStartOffset(Default=-1 => 0 for Forward, StrLenght for Backwards)"=w54) -> ("TextBeforeBlock"=w46:string, "found"=w44:bool, "BlockText"=w55:string, "BlockEnd(Outside)"=w53:i32)  [unwired: 9 in, 5 out]
    n11 = call "GDSString_PatternMatching.vi"("TextIn"=w46, "PatternMatchingStrings"=string[] ["}"] ("PatternMatchingString"), "Search Backwards"=TRUE) -> ("TextAfter"=w47:string, "Found"=w48:bool)  [unwired: 10 in, 5 out]
    n12 = Select(t=w47, s=w48, f=w46) -> (s? t:f=w45:string)
    n13 = Concatenate Strings(" " ("string"), w45) -> (w33:string)
    n14 = call "GDSString_PatternMatching.vi"("TextIn"=w33, "PatternMatchingStrings"=w34, "Search Backwards"=TRUE) -> ("IndexOfTheFoundPatternMatchingString"=w29:i32, "TextBefore"=w40:string, "Match"=w28:string, "TextAfter"=w41:string, "Found"=w42:bool)  [unwired: 10 in, 2 out]
    n15 = case shown="Default" w29 {
      selector: w29 -> [_ _ w89]
      tunnel: w55 -> [w59 w69 w136]
      tunnel: [_ _ w133] -> w52
      tunnel: w44 -> [_ _ w129]
      tunnel: [_ _ w128] -> w43
      tunnel: w42 -> [_ _ w127]
      tunnel: w41 -> [w57 w64 w101]
      tunnel: w40 -> [_ w66 w123]
      tunnel: w39 -> [_ _ w117]
      tunnel: w38 -> [w60 w61 w110]
      tunnel: [w58 w61 w107] -> w37
      tunnel: [_ _ w105] -> w36
      tunnel: [_ _ w95] -> w35
      tunnel: [w56 w67 w90] -> w31
      tunnel: w30 -> [_ w67 w90]
      tunnel: w28 -> [_ w65 _]
      tunnel: [_ w63 _] -> w27
      tunnel: [_ w62 _] -> w26
      frame 2 {
        # "namespace"
        n16 = call <vilib>:"Trim Whitespace.vi"("string"=w57) -> ("trimmed string"=w56:string)  [unwired: 1 in]
        n17 = Concatenate Strings(w60, w59) -> (w58:string)
      }
      frame 3, 4 {
        # "enums and Struct that aren't linked to a class ?!?!?"
        n18 = Format Into String(format string="%s %s\n{\n%s\n}", initial string=w66, w65, w64, w69) -> (resulting string=w68:string)  [unwired: 1 in, 1 out]
        n19 = call "GDSString_AttributeTextToAttributeType.vi"("Attribute,Struct,Enum-Text"=w68) -> ("Structs"=w63:T4[], "Enums"=w62:T1[])  [unwired: 7 in, 2 out]
      }
      frame Default {
        # "Class, Interface"
        n20 = while {
          shift-right: [w146] -> w100
          shift-left: w101 -> [w152]
          tunnel: [w145] -> w99 mode=indexing
          tunnel: [w144] -> w87 mode=indexing
          stop <- w149 continue-if-true
          # "Remove Generics"
          n21 = call "GDSString_FindCodeBlock.vi"("Text"=w152, "CodeBlockStartCharacter( { )"="<", "CodeBlockEndCharacter( } )"=">") -> ("TextBeforeBlock"=w148:string, "TextAfterBlock"=w147:string, "found"=w149:bool, "BlockText"=w145:string, "BlockStart(Outside)"=w144:i32)  [unwired: 8 in, 4 out]
          n22 = Concatenate Strings(w148, w147) -> (w146:string)
        }
        n23 = Index Array(array=w87) -> (element=w84:i32)  [unwired: 1 in]
        n24 = call "GDSString_FindWord.vi"("Text"=w100, "PatternMatchingDelimiter(\\s\\t\\r\\n)"="\\s\\t\\r\\n<" ("PatternMatchingDelimiter(\\s\\t\\r\\n)"), "Search Backwards"=FALSE) -> ("NextWord"=w73:string, "IndexAfterMatch(Or before when searching Backwards)"=w85:i32)  [unwired: 11 in, 4 out]
        n25 = while {
          shift-right: [w233] -> w72
          shift-left: w136 -> [w220]
          tunnel: [w232] -> w132 mode=indexing
          tunnel: [w231] -> w75 mode=indexing if=w221
          tunnel: w117 -> [w230]
          tunnel: [w227] -> w109 mode=indexing if=w225
          tunnel: [w226] -> w104 mode=indexing if=w225
          tunnel: w73 -> [w223]
          tunnel: w89 -> [w219]
          tunnel: w84 -> [_]
          stop <- w224 continue-if-true
          # "Loop through all {..} blocks inside this class or interface"
          n26 = case shown="Default" w219 {
            tunnel: [w240 w280] -> w233
            tunnel: [_ w279] -> w229
            tunnel: [w249 w275] -> w228
            tunnel: [w235 w276] -> w224
            tunnel: [w256 w278] -> w222
            tunnel: w220 -> [w239 w274]
            tunnel: [w246 _] -> w218
            tunnel: [w245 _] -> w217
            tunnel: [w244 _] -> w216
            frame 1 {
              # "Find Interface method"
              n27 = while {
                tunnel: w239 -> [w265]
                shift-right: [w264] -> _
                shift-left: 0 ("offset past match") -> [w263]
                tunnel: [w262] -> w254 mode=indexing if=w261
                stop <- w261 continue-if-true
                n28 = call "GDSString_FindCodeBlock.vi"("Text"=w265, "StringStartOffset(Default=-1 => 0 for Forward, StrLenght for Backwards)"=w263) -> ("found"=w261:bool, "BlockStart(Outside)"=w260:i32, "BlockEnd(Outside)"=w264:i32)  [unwired: 9 in, 6 out]
                n29 = Build Array(w260, w264) -> (w262:i32[])
              }
              n30 = while {
                tunnel: w239 -> [w272]
                shift-right: [w270] -> _
                shift-left: 0 ("offset past match") -> [w269]
                tunnel: [w268] -> w252 mode=indexing if=w267
                stop <- w267 continue-if-true
                n31 = call "GDSString_FindTextBasedCodeDocumenation.vi"("Text"=w272, "StringStartOffset(Default=-1 => 0 for Forward, StrLenght for Backwards)"=w269, "CommentHasToBeTheFirstItem(True)"=FALSE) -> ("Found"=w267:bool, "IndexBeforeDocument(Or after when searching Backwards)"=w271:i32, "IndexAfterDocument(Or before when searching Backwards)"=w270:i32)  [unwired: 12 in, 2 out]
                n32 = Build Array(w271, w270) -> (w268:i32[])
              }
              n33 = Match Pattern(string=w239, regular expression="^[\\s\\r\\n;]+$") -> (before substring=w242:string, after substring=w241:string)  [unwired: 1 in, 2 out]
              n34 = Concatenate Strings(w242, w241) -> (w238:string)
              n35 = Empty String/Path?(string/path=w238) -> (empty?=w236:bool)
              n36 = Not(x=w236) -> (.not. x?=w234:bool)
              n37 = Concatenate Strings(w238, ";" ("regular expression")) -> (w250:string)
              n38 = Build Array (concatenate)(w254, w252) -> (w253:i32[][])
              n39 = call "GDSString_PatternMatching.vi"("TextIn"=w250, "PatternMatchingStrings"=string[] [";"], "StringStartOffset(Default=-1 => 0 for Forward, StrLenght for Backwards)"=0 ("IndexAfterMatch(Or before when searching Backwards)"), "IgnoreMatchesWithinThesePositions"=w253) -> ("TextBefore"=w249:string, "TextAfter"=w240:string, "IndexAfterMatch(Or before when searching Backwards)"=w256:i32)  [unwired: 9 in, 4 out]
              n40 = Greater Or Equal To 0?(x=w256) -> (x >= 0?=w237:bool)
              n41 = call "GDSString_ParsePropertyMethod.vi"("PropertyMethodContent"=w249) -> ("SetProperty"=w244:T9, "GetProperty"=w245:T9)  [unwired: 9 in]
              n42 = Unbundle By Name(w244) -> ("Active"=w248:bool)
              n43 = Unbundle By Name(w245) -> ("Active"=w247:bool)
              n44 = Or(x=w247, y=w248) -> (x .or. y?=w246:bool)
              n45 = And(x=w237, y=w234) -> (x .and. y?=w235:bool)
            }
            frame Default {
              # "Find method block {...}"
              n46 = call "ConvertTextBasedCodeToLabVIEW_FixAbstractMethods.vi"("String"=w274) -> ("String 2"=w273:string)  [unwired: 10 in]
              n47 = while {
                tunnel: [w281] -> w280
                tunnel: [w288] -> w279
                tunnel: [w287] -> w278
                tunnel: [w282] -> w277
                tunnel: [w286] -> w276
                shift-right: [w283] -> _
                shift-left: w273 -> [w285]
                stop <- w284 continue-if-true
                # "Check for Java static{...} call (JNI )"
                n48 = call "GDSString_FindCodeBlock.vi"("Text"=w285) -> ("TextBeforeBlock"=w282:string, "TextAfterBlock"=w281:string, "found"=w286:bool, "BlockText"=w288:string, "BlockEnd(Outside)"=w287:i32)  [unwired: 10 in, 4 out]
                n49 = case shown="True" w286 {
                  tunnel: [FALSE w296] -> w284
                  tunnel: ["" ("regular expression") w291] -> w283
                  tunnel: w282 -> [_ w295]
                  tunnel: w281 -> [_ w292]
                  frame False {
                  }
                  frame True {
                    n50 = call "GDSString_FindWord.vi"("Text"=w295, "Search Backwards"=TRUE, "AllowedWords(PatternMatching)"=string[] ["static"], "ExactWord"=TRUE) -> ("IndexAfterMatches(Or before when searching Backwards)"=w298:i32[], "IndexAfterLastMatch(Or before when searching Backwards)"=w294:i32)  [unwired: 10 in, 4 out]
                    n51 = Empty Array?(array=w298) -> (empty?=w297:bool)
                    n52 = Not(x=w297) -> (.not. x?=w296:bool)
                    n53 = String Subset(string=w295, length (rest)=w294) -> (substring=w293:string)  [unwired: 1 in]
                    n54 = Concatenate Strings(w293, w292) -> (w291:string)
                  }
                }
              }
              n55 = call "GDSString_RemoveBaseMethodCallString.vi"("Method Call String"=w277) -> ("Base call Removed"=w275:string)  [unwired: 10 in]
            }
          }
          n56 = case shown="True" w224 {
            selector: w224 -> [_ w313]
            tunnel: [_ w317] -> w232
            tunnel: [_ w316] -> w231
            tunnel: w230 -> [_ w315]
            tunnel: w229 -> [_ w309]
            tunnel: w228 -> [_ w305]
            tunnel: [_ w314] -> w227
            tunnel: [_ w313] -> _
            tunnel: [_ w312] -> w226
            tunnel: [_ w311] -> w225
            tunnel: w223 -> [_ w310]
            tunnel: w222 -> [_ w308]
            tunnel: [_ w307] -> w221
            tunnel: w220 -> [_ w306]
            tunnel: w218 -> [_ w304]
            tunnel: w217 -> [_ w303]
            tunnel: w216 -> [_ w302]
            frame False {
            }
            frame True {
              n57 = case shown="True" w304 {
                tunnel: [w367 _] -> w317
                tunnel: [w363 w484] -> w316
                tunnel: w315 -> [w361 _]
                tunnel: [w359 _] -> w314
                tunnel: [w358 _] -> w312
                tunnel: [w357 _] -> w311
                tunnel: w310 -> [w356 _]
                tunnel: w309 -> [w340 _]
                tunnel: w308 -> [w339 _]
                tunnel: [w332 TRUE] -> w307
                tunnel: w306 -> [w331 _]
                tunnel: w305 -> [w327 w474]
                tunnel: w303 -> [_ w483]
                tunnel: w302 -> [_ w482]
                frame False {
                  w350 = TRUE ("Search Backwards")
                  n58 = while {
                    tunnel: w327 -> [w404]
                    shift-right: [w403] -> _
                    shift-left: 0 ("offset past match") -> [w402]
                    tunnel: [w401] -> w326 mode=indexing if=w400
                    stop <- w400 continue-if-true
                    n59 = call "GDSString_FindCodeBlock.vi"("Text"=w404, "StringStartOffset(Default=-1 => 0 for Forward, StrLenght for Backwards)"=w402, "CodeBlockStartCharacter( { )"="<", "CodeBlockEndCharacter( } )"=">") -> ("found"=w400:bool, "BlockStart(Outside)"=w397:i32, "BlockEnd(Outside)"=w403:i32)  [unwired: 7 in, 6 out]
                    n60 = Build Array(w397, w403) -> (w401:i32[])
                  }
                  n61 = call "GDSString_FindCodeBlock.vi"("Text"=w327, "CodeBlockStartCharacter( { )"="(", "CodeBlockEndCharacter( } )"=")", "Search Backwards"=TRUE) -> ("found"=w335:bool, "BlockText"=w362:string, "BlockStart(Outside)"=w360:i32)  [unwired: 7 in, 6 out]
                  n62 = Select(t=w360, s=w335, f=-1) -> (s? t:f=w342:i32)
                  n63 = call "GDSString_FindWord.vi"("Text"=w327, "StringStartOffset(Default=-1 => 0 for Forward, StrLenght for Backwards)"=w342, "Search Backwards"=w350, "AllowedWords(PatternMatching)"=string[] ["[~/*]+"], "GetNext-X_Words(1,-1=All)"=2 ("GetNext-X_Words(1)"), "IgnoreMatchesWithinThesePositions"=w326) -> ("NextWords"=w355:string[], "IndexAfterMatches(Or before when searching Backwards)"=w319:i32[], "IndexAfterLastMatch(Or before when searching Backwards)"=w325:i32)  [unwired: 8 in, 3 out]
                  n64 = Index Array(array=w355) -> (element #1=w324:string, element #2=w322:string)  [unwired: 2 in]
                  n65 = Search 1D Array(1D array=string[] ["class", "enum", "struct", "implements", ":"], element=w322) -> (index of element=w329:i32)  [unwired: 1 in]
                  n66 = case shown="-1" w329 {
                    tunnel: w327 -> [_ _ w384]
                    tunnel: w326 -> [_ _ w389]
                    tunnel: w325 -> [w370 w371 w388]
                    tunnel: [w370 w371 w375] -> w328
                    tunnel: w324 -> [w369 w373 _]
                    tunnel: [w369 w373 w379] -> w323
                    tunnel: w322 -> [w368 w372 _]
                    tunnel: [w368 w372 w377] -> w320
                    tunnel: w319 -> [_ _ _]
                    frame Default {
                    }
                    frame -1 {
                    }
                    frame 3, 4 {
                      w383 = TRUE ("Search Backwards")
                      w386 = 2 ("GetNext-X_Words(1)")
                      n67 = call "GDSString_FindWord.vi"("Text"=w384, "StringStartOffset(Default=-1 => 0 for Forward, StrLenght for Backwards)"=w388, "Search Backwards"=w383, "GetNext-X_Words(1,-1=All)"=w386, "IgnoreMatchesWithinThesePositions"=w389) -> ("NextWords"=w387:string[], "IndexAfterLastMatch(Or before when searching Backwards)"=w376:i32)  [unwired: 9 in, 4 out]
                      n68 = Index Array(array=w387) -> (element #1=w380:string, element #2=w378:string)  [unwired: 2 in]
                      n69 = call "GDSString_FindWord.vi"("Text"=w384, "StringStartOffset(Default=-1 => 0 for Forward, StrLenght for Backwards)"=w376, "Search Backwards"=w383, "GetNext-X_Words(1,-1=All)"=w386) -> ("NextWords"=w385:string[], "IndexAfterLastMatch(Or before when searching Backwards)"=w374:i32)  [unwired: 10 in, 4 out]
                      n70 = Equal?(x=w378, y="extends") -> (x = y?=w381:bool)
                      n71 = case shown="True" w381 {
                        tunnel: w385 -> [_ w396]
                        tunnel: w380 -> [w392 _]
                        tunnel: [w392 w395] -> w379
                        tunnel: w378 -> [w391 _]
                        tunnel: [w391 w394] -> w377
                        tunnel: w376 -> [w390 _]
                        tunnel: [w390 w393] -> w375
                        tunnel: w374 -> [_ w393]
                        frame False {
                        }
                        frame True {
                          n72 = Index Array(array=w396) -> (element #1=w395:string, element #2=w394:string)  [unwired: 2 in]
                        }
                      }
                    }
                  }
                  n73 = call "GDSString_FindWord.vi"("Text"=w327, "StringStartOffset(Default=-1 => 0 for Forward, StrLenght for Backwards)"=w328, "Search Backwards"=w350, "AllowedWords(PatternMatching)"=w361, "GetNext-X_Words(1,-1=All)"=-1, "ExactWord"=TRUE) -> ("NextWords"=w344:string[], "IndexAfterLastMatch(Or before when searching Backwards)"=w348:i32)  [unwired: 8 in, 4 out]
                  n74 = Empty Array?(array=w344) -> (empty?=w349:bool)
                  n75 = Equal?(x=w320, y="class") -> (x = y?=w333:bool)
                  n76 = Select(t=w328, s=w349, f=w348) -> (s? t:f=w338:i32)
                  n77 = call "GDSString_FindTextBasedCodeDocumenation.vi"("Text"=w327, "StringStartOffset(Default=-1 => 0 for Forward, StrLenght for Backwards)"=w338, "Search Backwards"=TRUE) -> ("Document"=w353:string, "Found"=w347:bool, "IndexBeforeDocument(Or after when searching Backwards)"=w346:i32)  [unwired: 12 in, 2 out]
                  n78 = Select(t=w346, s=w347, f=w338) -> (s? t:f=w345:i32)
                  n79 = Subtract(x=w339, y=w338) -> (x-y=w337:i32)
                  n80 = call <vilib>:"Trim Whitespace.vi"("string"=w340) -> ("trimmed string"=w336:string)  [unwired: 1 in]
                  n81 = case shown="-1" w329 {
                    tunnel: [w409 w453] -> w367
                    tunnel: [w438 _] -> w363
                    tunnel: w353 -> [w436 _]
                    tunnel: w345 -> [w434 w452]
                    tunnel: w327 -> [w433 w450]
                    tunnel: w336 -> [w413 w458]
                    tunnel: w356 -> [w431 _]
                    tunnel: w323 -> [w412 w457]
                    tunnel: w344 -> [w407 _]
                    tunnel: w362 -> [w427 _]
                    tunnel: w320 -> [w424 _]
                    tunnel: [_ w455] -> w359
                    tunnel: [_ w456] -> w357
                    tunnel: [_ w457] -> w358
                    tunnel: w331 -> [w421 _]
                    tunnel: w338 -> [w420 _]
                    tunnel: w337 -> [w419 _]
                    tunnel: w335 -> [w411 _]
                    tunnel: w333 -> [_ w456]
                    tunnel: [TRUE _] -> w332
                    tunnel: w326 -> [_ _]
                    tunnel: w320 -> [w405 _]
                    frame -1 {
                      w425 = GDSString_AccessScopeModifierType."public" ("DefaultAccessScope(Private)")
                      n82 = case shown="True" w411 {
                        tunnel: [w440 w446] -> w435
                        tunnel: w434 -> [_ w445]
                        tunnel: w433 -> [w440 w444]
                        tunnel: w407 -> [w439 w443]
                        tunnel: [w439 w442] -> w406
                        tunnel: w405 -> [_ w441]
                        frame False {
                        }
                        frame True {
                          n83 = String Subset(string=w444, length (rest)=w445) -> (substring=w446:string)  [unwired: 1 in]
                          n84 = Build Array (concatenate)(w441, w443) -> (w442:string[])
                        }
                      }
                      n85 = Equal?(x=w412, y=w431) -> (x = y?=w430:bool)
                      n86 = Select(t=w412, s=w430, f=w424) -> (s? t:f=w422:string)
                      n87 = call "GDSString_AttributeTextToAttributeType.vi"("MethodText"=w427, "DefaultAccessScope(Private)"=w425) -> ("Attributes"=w426:T5[])  [unwired: 6 in, 3 out]
                      n88 = call "GDSString_GetModifiers.vi"("Words"=w406) -> ("Array out"=w437:T3[], "AccessScope"=w432:T2)  [unwired: 8 in, 1 out]
                      n89 = call "GDSString_AttributeTextToAttributeType.vi"("MethodText"=w422, "DefaultAccessScope(Private)"=w425) -> ("Attributes"=w429:T5[])  [unwired: 6 in, 3 out]
                      n90 = String Subset(string=w421, offset (0)=w420, length (rest)=w419) -> (substring=w418:string)
                      n91 = Index Array(array=w429) -> (element=w428:T5)  [unwired: 1 in]
                      n92 = call <vilib>:"Trim Whitespace.vi"("string"=w418) -> ("trimmed string"=w414:string)  [unwired: 1 in]
                      n93 = case shown="True" w411 {
                        tunnel: [w449 _] -> w417
                        tunnel: [w448 _] -> w416
                        tunnel: w413 -> [w447 _]
                        frame False {
                          n94 = call "GDSString_ParsePropertyMethod.vi"("PropertyMethodContent"=w447) -> ("SetProperty"=w448:T9, "GetProperty"=w449:T9)  [unwired: 9 in]
                        }
                        frame True {
                        }
                      }
                      n95 = Bundle By Name(cluster=T8 {"ReturnType"={"Name"="", "DataType"=enum."UINT8", "ArrayDim"=0, "CtrlPath"=path "", "DataTypeString"="", "AccessScope"=enum."public", "InitialData"=variant}, "MethodName"="", "AccessScope"=enum."public", "Modifiers"=[], "MethodDocumentation"="", "MethodContent"="", "MethodArguments"=[], "GetProperty"={"Active"=FALSE, "AccessScope"=enum."public", "Code"=""}, "SetProperty"={"Active"=FALSE, "AccessScope"=enum."public", "Code"=""}}, "ReturnType"=w428, "MethodName"=w412, "AccessScope"=w432, "Modifiers"=w437, "MethodDocumentation"=w436, "MethodContent"=w414, "MethodArguments"=w426, "GetProperty"=w417, "SetProperty"=w416) -> (w438:T8)
                      n96 = call <vilib>:"Trim Whitespace.vi"("string"=w435) -> ("trimmed string"=w410:string)  [unwired: 1 in]
                      n97 = Concatenate Strings(w410, ";\n" ("string")) -> (w409:string)
                    }
                    frame Default {
                      n98 = Decrement(x=w452) -> (x-1=w451:i32)
                      n99 = Search/Split String(string=w450, offset (0)=w451) -> (substring before match=w461:string, match + rest of string=w459:string)  [unwired: 1 in, 1 out]
                      n100 = call <vilib>:"Trim Whitespace.vi"("string"=w461) -> ("trimmed string"=w454:string)  [unwired: 1 in]
                      n101 = Format Into String(format string="\n%s\n{\n%s\n}", w459, w458) -> (resulting string=w455:string)  [unwired: 2 in, 1 out]
                      n102 = case shown="False" w456 {
                        tunnel: w454 -> [w464 w465]
                        tunnel: w455 -> [w463 _]
                        tunnel: [w462 w465] -> w453
                        frame False {
                          n103 = Concatenate Strings(w464, w463) -> (w462:string)
                        }
                        frame True {
                        }
                      }
                    }
                  }
                }
                frame True {
                  w476 = T3[] [] items=["abstract", "static", "final", "synchronized", "strictfp", "async", "const", "event", "extern", "new", "native ", "override", "partial", "readonly", "sealed", "unsafe", "virtual", "volatile"] ("Modifiers")
                  # "public interface IMyInterface\n    {\n        int GetNumber(int FirstNumber);\n        int MyNumber { get; set; }\n        boolean IsEven();\n    }"
                  # "Interface class method.\nThis text is a Property Node Method\nE.g."
                  n104 = call "GDSString_FindCodeBlock.vi"("Text"=w474, "Search Backwards"=TRUE) -> ("TextBeforeBlock"=w473:string)  [unwired: 9 in, 8 out]
                  n105 = call "GDSString_FindWord.vi"("Text"=w473, "Search Backwards"=TRUE, "AllowedWords(PatternMatching)"=string[] ["[~/*]+"], "GetNext-X_Words(1,-1=All)"=2 ("GetNext-X_Words(1)")) -> ("NextWords"=w471:string[])  [unwired: 10 in, 5 out]
                  n106 = Index Array(array=w471) -> (element #1=w470:string, element #2=w469:string)  [unwired: 2 in]
                  n107 = call "GDSString_ParseDataTypeString.vi"("DefaultAccessScope(Private)"=GDSString_AccessScopeModifierType."public", "InputText"=w469) -> ("DataType"=w468:T5)  [unwired: 7 in, 2 out]
                  n108 = stacked-sequence {
                    frame #0 {
                    }
                  }
                  n109 = Bundle By Name(cluster=T8 {"ReturnType"={"Name"="", "DataType"=enum."UINT8", "ArrayDim"=0, "CtrlPath"=path "", "DataTypeString"="", "AccessScope"=enum."public", "InitialData"=variant}, "MethodName"="", "AccessScope"=enum."public", "Modifiers"=[], "MethodDocumentation"="", "MethodContent"="", "MethodArguments"=[], "GetProperty"={"Active"=FALSE, "AccessScope"=enum."public", "Code"=""}, "SetProperty"={"Active"=FALSE, "AccessScope"=enum."public", "Code"=""}}, "ReturnType"=w468, "MethodName"=w470, "AccessScope"=GDSString_AccessScopeModifierType."public", "Modifiers"=w476, "MethodDocumentation"="", "MethodContent"=w474, "MethodArguments"=T5[] [], "GetProperty"=w483, "SetProperty"=w482) -> (w484:T8)
                }
              }
            }
          }
        }
        n110 = Index Array(array=w99) -> (element=w82:string)  [unwired: 1 in]
        n111 = Equal?(x=w84, y=w85) -> (x = y?=w83:bool)
        n112 = Select(t=w82, s=w83, f="") -> (s? t:f=w80:string)
        n113 = call <vilib>:"Trim Whitespace.vi"("string"=w80) -> ("trimmed string"=w98:string)  [unwired: 1 in]
        n114 = Equal To 0?(x=w89) -> (x = 0?=w126:bool)
        n115 = Spreadsheet String To Array(delimiter (Tab)=",", format string="%s", spreadsheet string=w98, array type (2D Dbl)=string[] [] ("PatternMatchingString")) -> (array=w79:string[])
        n116 = Select(t=GDSString_ClassType."Class" ("ClassType"), s=w126, f=GDSString_ClassType."Interface" ("ClassType")) -> (s? t:f=w74:T11)
        n117 = String Subset(string=w100, offset (0)=w85) -> (substring=w121:string)  [unwired: 1 in]
        n118 = case shown="\"Class\"" w74 {
          tunnel: [GDSString_AccessScopeModifierType."public" ("AccessScope") w209] -> w134
          tunnel: w117 -> [_ w214]
          tunnel: w123 -> [_ w213]
          tunnel: [-1 ("IndexAfterMatch(Or before when searching Backwards)") w212] -> w122
          tunnel: [_ w208] -> w115
          frame "Undefined", Default {
          }
          frame "Class" {
            n119 = call "GDSString_FindWord.vi"("Text"=w213, "Search Backwards"=TRUE, "AllowedWords(PatternMatching)"=w214, "GetNext-X_Words(1,-1=All)"=-1) -> ("IndexAfterMatch(Or before when searching Backwards)"=w212:i32, "NextWords"=w210:string[])  [unwired: 10 in, 4 out]
            n120 = call "GDSString_GetModifiers.vi"("Words"=w210) -> ("Array out"=w208:T3[], "AccessScope"=w209:T2)  [unwired: 8 in, 1 out]
          }
        }
        n121 = call "GDSString_PatternMatching.vi"("TextIn"=w121, "PatternMatchingStrings"=string[] [":", "extends ", "implements "]) -> ("IndexOfTheFoundPatternMatchingString"=w118:i32, "TextAfter"=w114:string, "Found"=w119:bool)  [unwired: 11 in, 4 out]
        n122 = for {
          tunnel: w79 -> [w142] mode=indexing
          tunnel: [w141] -> w78 mode=indexing
          n123 = call <vilib>:"Trim Whitespace.vi"("string"=w142) -> ("trimmed string"=w141:string)  [unwired: 1 in]
        }
        n124 = case shown="False" w119 {
          tunnel: w118 -> [_ w160]
          tunnel: w114 -> [_ w159]
          tunnel: T10 {"ClassName"="", "ClassType"=enum."Undefined"} ("Parent") -> [_ w158]
          tunnel: [_ w157] -> w112
          frame False {
          }
          frame True {
            n125 = case shown="0, Default" w160 {
              selector: w160 -> [_ w189]
              tunnel: w159 -> [w168 w190]
              tunnel: w158 -> [w161 w175]
              tunnel: [w162 w181] -> w157
              frame 0, Default {
                # "c# way of inheritens or interface"
                n126 = call <vilib>:"Trim Whitespace.vi"("string"=w168) -> ("trimmed string"=w165:string)  [unwired: 1 in]
                n127 = Spreadsheet String To Array(delimiter (Tab)=",", format string="%s", spreadsheet string=w165, array type (2D Dbl)=string[] [] ("PatternMatchingString")) -> (array=w164:string[])
                n128 = for {
                  tunnel: w164 -> [w171] mode=indexing
                  tunnel: w161 -> [w172]
                  tunnel: [w170] -> w162 mode=indexing
                  n129 = call <vilib>:"Trim Whitespace.vi"("string"=w171) -> ("trimmed string"=w169:string)  [unwired: 1 in]
                  n130 = Bundle(cluster=w172, "ClassName"=w169) -> (w170:T10)  [unwired: 1 in]
                }
              }
              frame 1, 2 {
                # "JAVA style of inheritance and interface"
                n131 = case shown="1, Default" w189 {
                  tunnel: w190 -> [w204 w205]
                  tunnel: [w202 _] -> w183
                  tunnel: [w201 w205] -> w173
                  frame 1, Default {
                    n132 = Match Pattern(string=w204, regular expression="[\\s]+implements[\\s]+") -> (before substring=w202:string, after substring=w201:string)  [unwired: 1 in, 2 out]
                  }
                  frame 2 {
                  }
                }
                n133 = call <vilib>:"Trim Whitespace.vi"("string"=w183) -> ("trimmed string"=w186:string)  [unwired: 1 in]
                n134 = call <vilib>:"Trim Whitespace.vi"("string"=w173) -> ("trimmed string"=w178:string)  [unwired: 1 in]
                n135 = Spreadsheet String To Array(delimiter (Tab)=",", format string="%s", spreadsheet string=w186, array type (2D Dbl)=string[] [] ("PatternMatchingString")) -> (array=w185:string[])
                n136 = Spreadsheet String To Array(delimiter (Tab)=",", format string="%s", spreadsheet string=w178, array type (2D Dbl)=string[] [] ("PatternMatchingString")) -> (array=w179:string[])
                n137 = for {
                  tunnel: w179 -> [w194] mode=indexing
                  tunnel: w175 -> [w195]
                  tunnel: [w193] -> w174 mode=indexing
                  n138 = call <vilib>:"Trim Whitespace.vi"("string"=w194) -> ("trimmed string"=w192:string)  [unwired: 1 in]
                  n139 = Bundle(cluster=w195, "ClassName"=w192, "ClassType"=GDSString_ClassType."Interface") -> (w193:T10)
                }
                n140 = for {
                  tunnel: w185 -> [w199] mode=indexing
                  tunnel: w175 -> [w200]
                  tunnel: [w198] -> w182 mode=indexing
                  n141 = call <vilib>:"Trim Whitespace.vi"("string"=w199) -> ("trimmed string"=w197:string)  [unwired: 1 in]
                  n142 = Bundle(cluster=w200, "ClassName"=w197, "ClassType"=GDSString_ClassType."Class") -> (w198:T10)
                }
                n143 = Build Array (concatenate)(w182, w174) -> (w181:T10[])
              }
            }
          }
        }
        n144 = call "GDSString_FindTextBasedCodeDocumenation.vi"("Text"=w123, "StringStartOffset(Default=-1 => 0 for Forward, StrLenght for Backwards)"=w122, "Search Backwards"=TRUE) -> ("Document"=w130:string)  [unwired: 12 in, 4 out]
        n145 = case shown="\"\"" w90 {
          tunnel: [GDSString_ClassOwnerType."Package/NameSpace" ("OwnerType") _] -> w91
          frame Default {
          }
          frame "" {
          }
        }
        n146 = Concatenate Strings(w132, w72) -> (w111:string)
        n147 = Concatenate Strings(w109) -> (w106:string)
        n148 = call <vilib>:"Trim Whitespace.vi"("string"=w111) -> ("trimmed string"=w94:string)  [unwired: 1 in]
        n149 = Empty String/Path?(string/path=w106) -> (empty?=w108:bool)
        n150 = call "GDSString_AttributeTextToAttributeType.vi"("RemoveAttributesWithEmptynames(False)"=TRUE, "Attribute,Struct,Enum-Text"=w94) -> ("Structs"=w92:T4[], "Enums"=w93:T1[], "Attributes"=w77:T5[])  [unwired: 6 in, 1 out]
        n151 = case shown="Default" w74 {
          tunnel: w77 -> [w137 w140]
          tunnel: [w137 w139] -> w76
          tunnel: w75 -> [_ w138]
          frame "Interface" {
          }
          frame Default {
            n152 = call "CommonVIs_UpdateAttributesFromPropertyMethods.vi"("Methods"=w138, "Attributes in"=w140) -> ("Attributes out"=w139:T5[])  [unwired: 9 in]
          }
        }
        n153 = Bundle(cluster=cluster{"Owner":string, "Nested":string[]} {"Owner"="", "Nested"=[]}, "Owner"=w73, "Nested"=w104) -> (w105:cluster{"Owner":string, "Nested":string[]})
        n154 = Empty Array?(array=w104) -> (empty?=w103:bool)
        n155 = case shown="True" w108 {
          tunnel: w110 -> [w155 w156]
          tunnel: [w154 w156] -> w107
          tunnel: w106 -> [w153 _]
          frame False {
            n156 = Concatenate Strings(w155, w153) -> (w154:string)
          }
          frame True {
          }
        }
        n157 = Bundle By Name(cluster=T7 {"ClassName"="", "AccessScope"=enum."public", "Modifiers"=[], "ClassDocumentation"="", "Methods"=[], "ParentClasses"=[], "ClassType"=enum."Undefined", "Owner"="", "OwnerType"=enum."NoOwner", "Generics"=[], "Attributes"=[], "Enums"=[], "Structs"=[]} ("Class"), "Owner"=w90, "OwnerType"=w91, "Generics"=w78, "ClassName"=w73, "ClassType"=w74, "AccessScope"=w134, "Modifiers"=w115, "ClassDocumentation"=w130, "ParentClasses"=w112, "Attributes"=w76, "Enums"=w93, "Structs"=w92, "Methods"=w75) -> (w133:T7)
        n158 = Not(x=w103) -> (.not. x?=w95:bool)
        n159 = And(x=w127, y=w129) -> (x .and. y?=w128:bool)
      }
    }
  }
  "StructsOusideClass" <- w11
  "EnumsOusideClass" <- w12
  n160 = for {
    tunnel: w19 -> [w487] mode=indexing
    tunnel: [w486] -> w18 mode=indexing
    n161 = Unbundle By Name(w487) -> ("ClassName"=w486:string)
  }
  n162 = for {
    tunnel: w20 -> [w493] mode=indexing
    shift-right: [w488] -> w17
    shift-left: w19 -> [w491]
    tunnel: w18 -> [w490]
    n163 = Unbundle(w493) -> ("Owner"=w489:string, "Nested"=w492:string[])
    n164 = for {
      tunnel: w492 -> [w499] mode=indexing
      shift-right: [w494] -> w488
      shift-left: w491 -> [w497]
      tunnel: w490 -> [w498]
      tunnel: w489 -> [w495]
      n165 = Search 1D Array(1D array=w498, element=w499) -> (index of element=w496:i32)  [unwired: 1 in]
      n166 = in-place {
        in-place-border: w495 -> [w501]
        n167 = in-place-array #1(w497, w496) -> (w503:T7)
        n168 = Bundle By Name(cluster=w503, "Owner"=w501, "OwnerType"=GDSString_ClassOwnerType."Class") -> (w502:T7)
        n169 = in-place-array #1(w502) -> (w494:T7[])  [unwired: 1 out]
      }
    }
  }
  "Classes" <- w17
  "error out" <- "error in (no error)"
